vi "Write Data Folder.vi"(8 "error in (no error)":errorcluster, 10 "Data Folder":path, 11 "Project Store-INI in":refnum<class "Project Store-INI.lvclass">) -> (0 "error out":errorcluster, 3 "Project Store-INI out":refnum<class "Project Store-INI.lvclass">)   [LabVIEW 2024, in "Project Store-INI.lvclass"]
doc: "Writes one field of this class's private data. Generated by lvai_create_accessors from the class private data control."
uses:
  Project Store-INI.lvclass
  Project Store-INI.lvclass/Project Store-INI.ctl
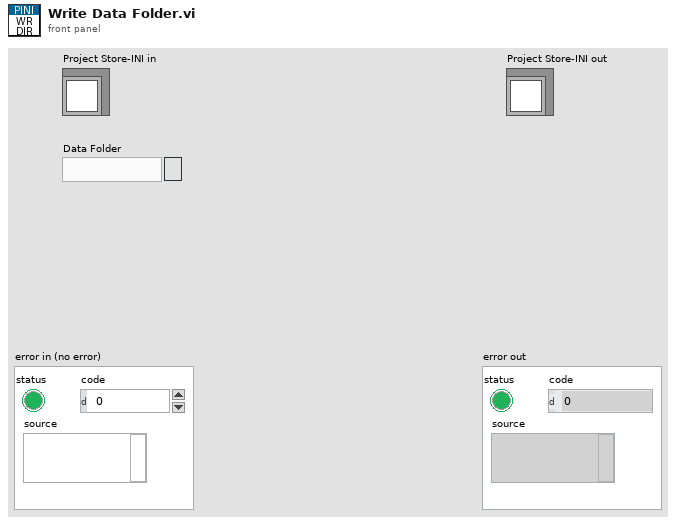
[diagram p1: front panel]
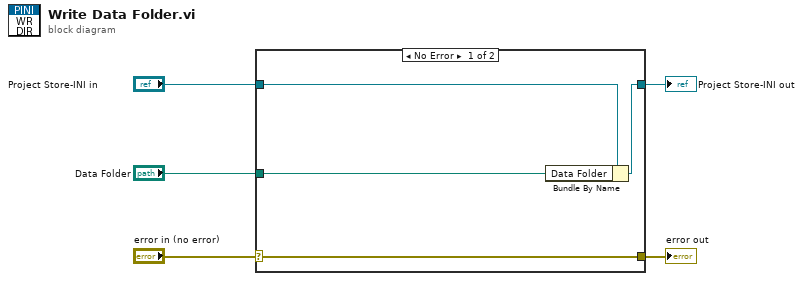
[diagram p0: block diagram]
diagram:
  n1 = case shown="No Error" "error in (no error)" {
    selector: "error in (no error)" -> [w9 w10]
    tunnel: [w9 w10] -> w4
    tunnel: [w7 w11] -> w2
    tunnel: "Project Store-INI in" -> [w8 w11]
    tunnel: "Data Folder" -> [w6 _]
    frame No Error {
      n2 = Bundle By Name(cluster=w8, "Data Folder"=w6) -> (w7:refnum<class "Project Store-INI.lvclass">)
    }
    frame Error {
    }
  }
  "error out" <- w4
  "Project Store-INI out" <- w2
